vi "Init.vi"(8 "error in (no error)":errorcluster, 10 "ServoDrive.lvclass":refnum<class "ServoDrive.lvclass">, 11 "Motor in":refnum<class "Motor.lvclass">) -> (0 "error out":errorcluster, 3 "Motor out":refnum<class "Motor.lvclass">)   [LabVIEW 2021, in "Motor.lvclass"]
uses:
  Motor.lvclass
  ServoDrive/ServoDrive.lvclass
  Motor.lvclass/Motor.ctl
  AnalogInput/AnalogInput.lvclass
  AnalogOutput/AnalogOutput.lvclass
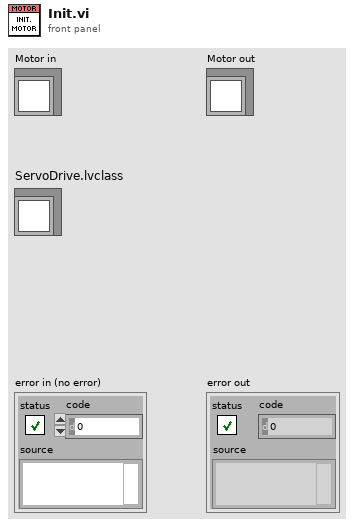
[diagram p1: front panel]
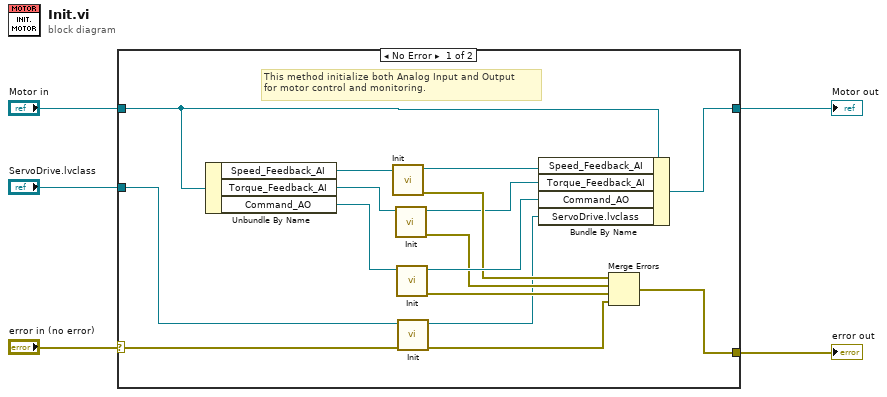
[diagram p0: block diagram]
diagram:
  n1 = case shown="No Error" "error in (no error)" {
    selector: "error in (no error)" -> [w9 w23]
    tunnel: [w16 w23] -> w4
    tunnel: [w19 w22] -> w2
    tunnel: "Motor in" -> [w7 w22]
    tunnel: "ServoDrive.lvclass" -> [w10 _]
    frame No Error {
      # "This method initialize both Analog Input and Output\nfor motor control and monitoring."
      n2 = Unbundle By Name(w7) -> ("Speed_Feedback_AI"=w15:refnum<class "AnalogInput.lvclass">, "Torque_Feedback_AI"=w13:refnum<class "AnalogInput.lvclass">, "Command_AO"=w14:refnum<class "AnalogOutput.lvclass">)
      n3 = call-dynamic "Init.vi"("AnalogInput in"=w15) -> ("error out"=w18:errorcluster, "AnalogInput out"=w21:refnum<class "AnalogInput.lvclass">)  [unwired: 9 in]
      n4 = call-dynamic "Init.vi"("AnalogInput in"=w13) -> ("error out"=w12:errorcluster, "AnalogInput out"=w11:refnum<class "AnalogInput.lvclass">)  [unwired: 9 in]
      n5 = call-dynamic "Init.vi"("AnalogOutput in"=w14) -> ("error out"=w17:errorcluster, "AnalogOutput out"=w20:refnum<class "AnalogOutput.lvclass">)  [unwired: 9 in]
      n6 = call-dynamic "Init.vi"("error in (no error)"=w9, "ServoDrive in"=w10) -> ("error out"=w8:errorcluster, "ServoDrive out"=w6:refnum<class "ServoDrive.lvclass">)  [unwired: 8 in]
      n7 = Bundle By Name(cluster=w7, "Speed_Feedback_AI"=w21, "Torque_Feedback_AI"=w11, "Command_AO"=w20, "ServoDrive.lvclass"=w6) -> (w19:refnum<class "Motor.lvclass">)
      n8 = Merge Errors(w18, w12, w17, w8) -> (w16:errorcluster)
    }
    frame Error {
    }
  }
  "error out" <- w4
  "Motor out" <- w2
